vi "to_json.vi"(8 "error in":errorcluster, 11 "include in":refnum<class "include.lvclass">) -> (0 "error out":errorcluster, 2 "json":string, 3 "include out":refnum<class "include.lvclass">, 4 "Not Default":bool)   [LabVIEW 2020, in "nominal types.lvlib" / "channelFilter.lvlib" / "include.lvclass"]
uses:
  include.lvclass
  include.lvclass/include.ctl
  b423daf5-c2a3-4c24-a941-a75b541187cf.vi
  <vilib>/JDP Science/JSONtext/support/Format JSON Array Text.vi
  <vilib>/JDP Science/JSONtext/Variant to JSON Text.vi
  <vilib>/JDP Science/JSONtext/support/Format JSON Object.vi
  <vilib>/JDP Science/JSONtext/LVClass Serializer/JSONtext LVClass Serializer.lvclass
  filterTypes/filterTypes.lvclass
  <vilib>/JDP Science/JSONtext/JSONtext.lvlib
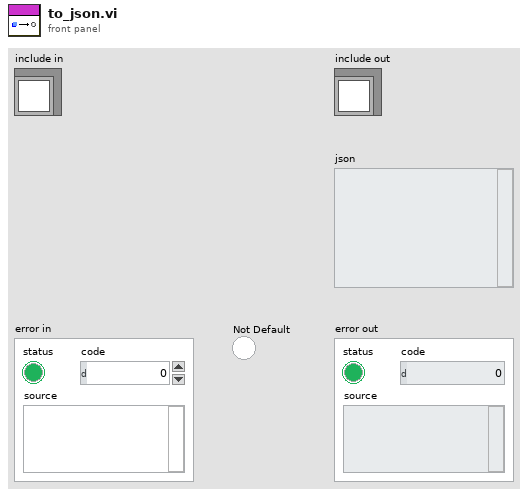
[diagram p1: front panel]
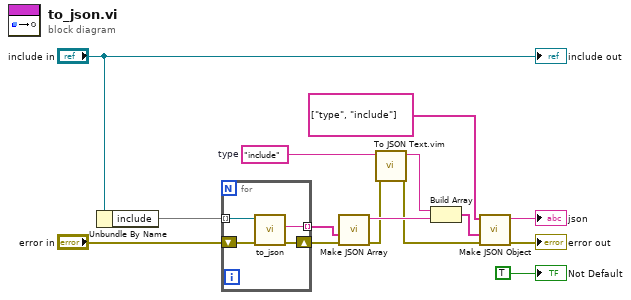
[diagram p0: block diagram]
diagram:
  w9 = "include"  # type
  n1 = Unbundle By Name("include in") -> ("include"=w14:set{refnum<class "filterTypes.lvclass">})
  n2 = for {
    tunnel: w14 -> [w17] mode=indexing
    tunnel: [w19] -> w12 mode=indexing
    shift-right: [w18] -> w11
    shift-left: "error in" -> [w16]
    n3 = call-dynamic "to_json.vi"("error in"=w16, "filterTypes in"=w17) -> ("error out"=w18:errorcluster, "json"=w19:string)  [unwired: 6 in, 2 out]
  }
  n4 = call <vilib>:"Make JSON Array.vi"("error in (no error)"=w11, "JSON Elements"=w12) -> ("error out"=w3:errorcluster, "<JSON>"=w8:string)  [unwired: 8 in]
  n5 = call "To JSON Text.vim"("error in (no error)"=w3, "Anything"=w9) -> ("error out"=w2:errorcluster, "<JSON>"=w4:string)  [unwired: 8 in]
  n6 = Build Array(w4, w8) -> (w7:string[])
  n7 = call <vilib>:"Make JSON Object.vi"("error in (no error)"=w2, "JSON Items"=w7, "Item Names"=string[] ["type", "include"]) -> ("error out"=→"error out":errorcluster, "<JSON>"=→"json":string)  [unwired: 7 in]
  "include out" <- "include in"
  "Not Default" <- TRUE ("Not Default")
